vi "PathPlanner_PathFinding_IsNewPathAvailable.vi"(8 "error in (no error)":errorcluster) -> (0 "error out":errorcluster, 3 "New Path Available":bool)   [LabVIEW 2019, in "PathPlanner24.lvlib"]
doc: "DOCUMENTATION NOT COMPLETE YET."
uses:
  PathPlanner24.lvlib
  PathPlanner_PathFinder_Globals.vi
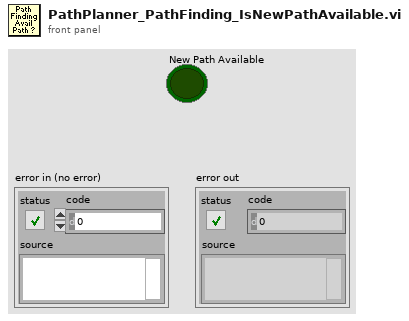
[diagram p1: front panel]
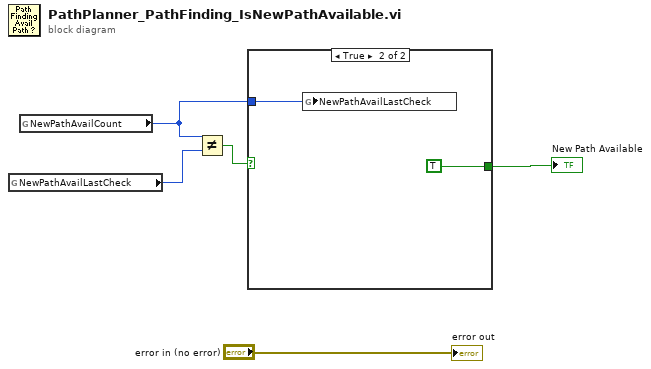
[diagram p0: block diagram]
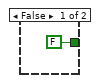
[diagram p2: hidden frame]
diagram:
  n1 = global read "PathPlanner_PathFinder_Globals.vi" "NewPathAvailLastCheck"() -> (w5:i32)
  n2 = global read "PathPlanner_PathFinder_Globals.vi" "NewPathAvailCount"() -> (w3:i32)
  n3 = Not Equal?(x=w3, y=w5) -> (x != y?=w4:bool)
  n4 = case shown="True" w4 {
    tunnel: w3 -> [_ w8]
    tunnel: [FALSE TRUE] -> w2
    frame False {
    }
    frame True {
      n5 = global write "PathPlanner_PathFinder_Globals.vi" "NewPathAvailLastCheck"(w8) -> ()
    }
  }
  "New Path Available" <- w2
  "error out" <- "error in (no error)"
